vi "CircleMath.vi"(1 "Target Heading":dbl, 2 "Current Heading":dbl) -> (0 "Delta Heading":dbl)   [LabVIEW 2014]
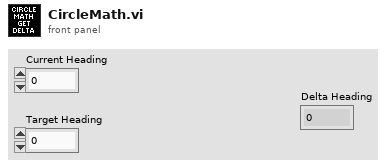
[diagram p1: front panel]
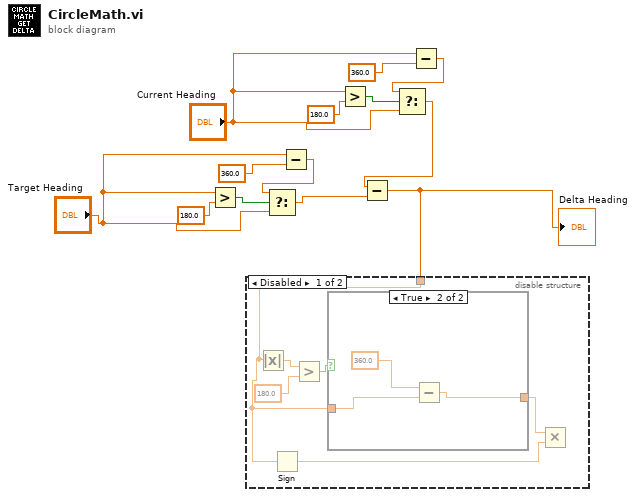
[diagram p0: block diagram]
diagram:
  n1 = Greater?(x="Target Heading", y=180.0) -> (0:w5:bool)
  n2 = Subtract(x="Target Heading", y=360.0) -> (x-y=w4:dbl)
  n3 = Select(t=w4, s=w5, f="Target Heading") -> (s? t:f=w2:dbl)
  n4 = Greater?(x="Current Heading", y=180.0) -> (0:w12:bool)
  n5 = Subtract(x="Current Heading", y=360.0) -> (x-y=w11:dbl)
  n6 = Select(t=w11, s=w12, f="Current Heading") -> (s? t:f=w10:dbl)
  n7 = Subtract(x=w10, y=w2) -> (x-y=w7:dbl)
  "Delta Heading" <- w7
  n8 = disable-structure shown="Disabled" {
    disable-tunnel: w7 -> [w15 _]
    frame Disabled {
      n9 = Absolute Value(x=w15) -> (abs(x)=w19:dbl)
      n10 = Sign(1:w15) -> (0:w14:dbl)
      n11 = Greater?(x=w19, y=180.0) -> (0:w17:bool)
      n12 = case shown="True" w17 {
        tunnel: w15 -> [w20 w22]
        tunnel: [w20 w21] -> w16
        frame False {
        }
        frame True {
          n13 = Subtract(x=360.0, y=w22) -> (x-y=w21:dbl)
        }
      }
      n14 = Multiply(x=w16, y=w14) -> ()  [unwired: 1 out]
    }
    frame Enabled {
    }
  }
